vi "SMTP Email Register Recipients.vi"(4 "error in (no error)":errorcluster caption="entrée d'erreur (pas d'erreur)", 6 "recipients":string[](array[string]) caption="destinataires", 7 "smtp session":T1 caption="session smtp") -> (0 "error out":errorcluster caption="sortie d'erreur", 2 "invalid recipients":string[](array[string]) caption="destinataires non valides", 3 "smtp session out":T1 caption="session smtp en sortie")   [LabVIEW 2022 SP3, in "Copie de NI_SMTPEmail.lvlib"]
doc: "Ce VI enregistre les destinataires du mail avec le serveur SMTP.\n\nSession SMTP : descripteur de la connexion SMTP du serveur SMTP.\n\nDestinataires : Un tableau de chaînes représentant les adresses e-mail des boîtes aux lettres des destinataires de l'e-mail. Remarquez que si un (ou plusieurs) des destinataires ne sont pas reconnus, le VI conservera l'enregistrement des destinataires restants jusqu'à ce que le tableau soit sollicité.\n\nDestinataires non valides : un tableau de destinataires non reconnus.\n\nSortie d'erreur : le cluster sortie d'erreur peut contenir une chaîne d'erreur même si le booléen état est FAUX. Cela arrive dans le cas de l'erreur 550 (destinataire non reconnu) en provenance du serveur SMTP."
uses:
  Copie de NI_SMTPEmail.lvlib
  SMTP Email Session.ctl
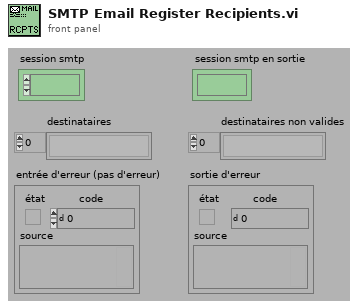
[diagram p1: front panel]
types:
  T1 = typedef "Copie de NI_SMTPEmail.lvlib/SMTP Email Session.ctl" = refnum<k1>
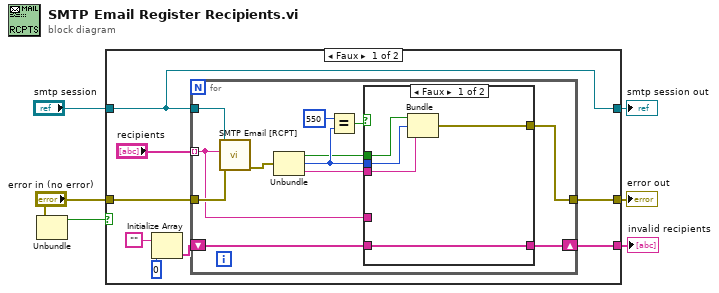
[diagram p0: block diagram]
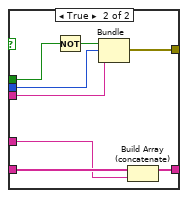
[diagram p2: hidden frame]
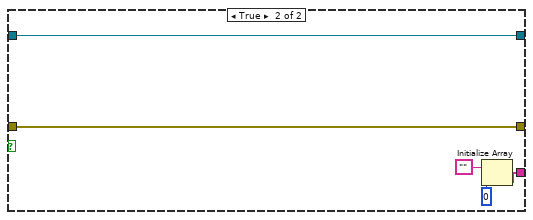
[diagram p3: hidden frame]
diagram:
  n1 = Unbundle("error in (no error)") -> ("status"=w5:bool)  [unwired: 2 out]
  n2 = case shown="Faux" w5 {
    tunnel: "error in (no error)" -> [w14 w44]
    tunnel: [w13 w44] -> w4
    tunnel: "smtp session" -> [w7 w43]
    tunnel: [w7 w43] -> w3
    tunnel: [w11 w40] -> w1
    frame False {
      n3 = Initialize Array("", 0) -> (w10:string[])
      n4 = for {
        tunnel: w14 -> [w26]
        tunnel: [w23] -> w13
        tunnel: w7 -> [w18]
        tunnel: "recipients" -> [w15] mode=indexing
        shift-right: [w16] -> w11
        shift-left: w10 -> [w17]
        n5 = call "SMTP Email [RCPT].vi"("error in (no error)"=w26, "address"=w15, "smtp session"=w18) -> ("error out"=w19:errorcluster)  [unwired: 1 in, 3 out]
        n6 = Unbundle(w19) -> ("status"=w20:bool, "code"=w21:i32, "source"=w22:string)
        n7 = Equal?(x=550, y=w21) -> (x = y?=w24:bool)
        n8 = case shown="Faux" w24 {
          tunnel: [w29 w39] -> w23
          tunnel: w22 -> [w30 w35]
          tunnel: w21 -> [w31 w38]
          tunnel: w20 -> [w28 w36]
          tunnel: w17 -> [w27 w34]
          tunnel: w15 -> [_ w33]
          tunnel: [w27 w32] -> w16
          frame False {
            n9 = Bundle("status"=w28, "code"=w31, "source"=w30) -> (w29:errorcluster)  [unwired: 1 in]
          }
          frame True {
            n10 = Not(x=w36) -> (.not. x?=w37:bool)
            n11 = Bundle(w37, "code"=w38, "source"=w35) -> (w39:cluster{bool, "code":i32, "source":string})  [unwired: 1 in]
            n12 = Build Array (concatenate)(w34, w33) -> (w32:string[])
          }
        }
      }
    }
    frame True {
      n13 = Initialize Array("", 0) -> (w40:string[])
    }
  }
  "smtp session out" <- w3
  "error out" <- w4
  "invalid recipients" <- w1
